vi "Toast From XML.vi"(8 "error in":errorcluster) -> (0 "error out":errorcluster, 3 "Toast XML":string)   [LabVIEW 2026]
doc: "Display a Windows toast from an XML string and receive its reply as a LabVIEW User Event. Click Send and inspect Activation.Arguments and the Reason entry in Activation.User Inputs. Press Stop to release the service and XML source. See the XML example guide for the input and expected results."
uses:
  ToastNotification/Activation.ctl
  ToastNotification/Argument.ctl
  PlugIns/UserEventActivationHandler/UserEventActivationHandler.lvclass
  PlugIns/UserEventActivationHandler/UserEventActivationHandler.lvclass/UserEventActivationHandler.ctl
  PlugIns/UserEventActivationHandler/Read Event Ref.vi
  ToastFromXML/ToastFromXML.lvclass
  ToastFromXML/Create ToastFromXML.vi
  ToastService/ToastService.lvclass
  ToastNotification/ToastNotification.lvlib
panel:
  out "error":errorcluster
  out "Activation":T1
  in  "stop":bool
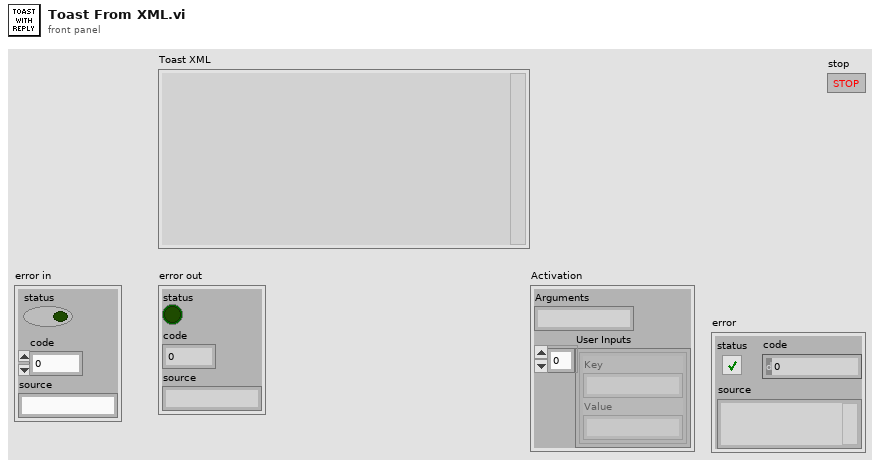
[diagram p1: front panel]
types:
  T1 = typedef "ToastNotification.lvlib/Activation.ctl" = cluster{"Arguments":string, "User Inputs":T2[]}
  T2 = typedef "ToastNotification.lvlib/Argument.ctl" = cluster{"Key":string, "Value":string}
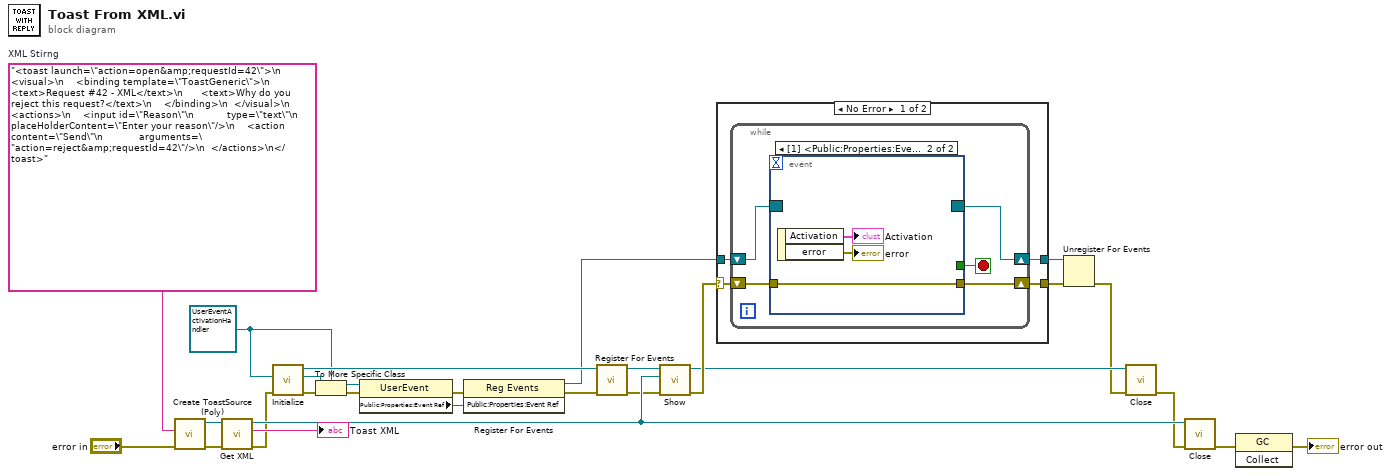
[diagram p0: block diagram]
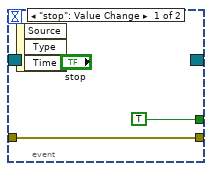
[diagram p2: hidden frame]
diagram:
  w2 = "<toast launch=\"action=open&amp;requestId=42\">\n  <visual>\n    <binding template=\"ToastGeneric\">\n      <text>Request #42 - XML</text>\n      <text>Why do you reject this request?</text>\n    </binding>\n  </visual>\n  <actions>\n    <input id=\"Reason\"\n           type=\"text\"\n           placeHolderContent=\"Enter your reason\"/>\n    <action content=\"Send\"\n            arguments=\"action=reject&amp;requestId=42\"/>\n  </actions>\n</toast>"  # XML Stirng
  w12 = refnum<class "UserEventActivationHandler.lvclass"> refnum
  n1 = call-poly "Create ToastSource (Poly).vi"("error in (no error)"="error in", "XML Stirng"=w2) -> ("error out"=w26:errorcluster, "ToastFromXML out"=w1:refnum<class "ToastFromXML.lvclass">)  [unwired: 8 in]
  n2 = call-dynamic "Get XML.vi"("error in (no error)"=w26, "ToastFromXML in"=w1) -> ("error out"=w23:errorcluster, "GetContent"=→"Toast XML":string, "ToastFromXML out"=w24:refnum<class "ToastFromXML.lvclass">)  [unwired: 7 in]
  n3 = call "Initialize.vi"("error in (no error)"=w23, "ActivationHandler in"=w12) -> ("error out"=w21:errorcluster, "ActivationHandler out"=w11:refnum<class "UserEventActivationHandler.lvclass">, "ToastService out"=w19:refnum<class "ToastService.lvclass">)  [unwired: 7 in]
  n4 = To More Specific Class(target class=w12, reference=w11, error in=w21) -> (specific class reference=w9:refnum<class "UserEventActivationHandler.lvclass">, error out=w13:errorcluster)
  n5 = property class="UserEvent"(reference=w9, error in=w13) -> (error out=w10:errorcluster, "Public:Properties:Event Ref"=w7:refnum<user-event>)  [unwired: 1 out]
  n6 = register-events(error in=w10, w7) -> (reference out=w6:refnum<event-registration>, error out=w8:errorcluster)  [unwired: 1 in]
  n7 = call "Register For Events.vi"("error in (no error)"=w8, "ToastService in"=w19) -> ("error out"=w20:errorcluster, "ToastService out"=w18:refnum<class "ToastService.lvclass">)  [unwired: 8 in]
  n8 = call "Show.vi"("error in (no error)"=w20, "ToastSource in"=w24, "ToastService in"=w18) -> ("error out"=w17:errorcluster, "ToastService out"=w16:refnum<class "ToastService.lvclass">)  [unwired: 7 in]
  n9 = case shown="No Error" w17 {
    selector: w17 -> [w31 w42]
    tunnel: [w30 w42] -> w5
    tunnel: w6 -> [w29 w43]
    tunnel: [w28 w43] -> w3
    frame No Error {
      n10 = while {
        shift-right: [w35] -> w30
        shift-left: w31 -> [w36]
        shift-right: [w33] -> w28
        shift-left: w29 -> [w34]
        stop <- w32 stop-if-true
        n11 = event shown="[1] <Public:Properties:Event Ref>: User Event" {
          selector: w34 -> [_ _]
          dyn-events: [_ _] -> w33
          timeout: _ -> [_ _]
          tunnel: [w38 w41] -> w35
          tunnel: w36 -> [w38 w41]
          tunnel: [TRUE _] -> w32
          event "stop": Value Change {
            n12 = event-data() -> ()  [unwired: 1 in, 3 out]
          }
          event User Event {
            n13 = event-data() -> ("Activation"=→"Activation":T1, "error"=→"error":errorcluster)  [unwired: 1 in]
          }
        }
      }
    }
    frame Error {
    }
  }
  n14 = Unregister For Events(event registration refnum=w3, error in=w5) -> (error out=w4:errorcluster)
  n15 = call "Close.vi"("error in (no error)"=w4, "ToastService in"=w16) -> ("error out"=w22:errorcluster)  [unwired: 9 in]
  n16 = call-dynamic "Close.vi"("error in (no error)"=w22, "ToastFromXML in"=w24) -> ("error out"=w15:errorcluster)  [unwired: 9 in]
  n17 = invoke class="GC" method="Collect"(error in=w15) -> (error out=→"error out":errorcluster)  [unwired: 2 in, 2 out]
